vi "MainLUT.vi"(9 "Sample Number":u32, 10 "Run ID":string="run-1791786455269", 11 "LUT Selector":T3) -> (0 "error out":errorcluster, 3 "Sample":T1={"axis info"={"Horizontal"=0, "Vertical"=0, "Scrolling"=0}, "button info"={"button 1"=FALSE, "button 2"=FALSE, "button 3"=FALSE, "button 4"=FALSE}, "Relative Time (User Event)"=0.0, "Sample Number"=0, "Relative Time (Frame 0)"=0.0, "key mode"=enum."ABSOLUTE", "Frame Number"=0, "Keyboard KeysPressed"=[], "Keyboard No Op"=FALSE})   [LabVIEW 2026, in "dependencies.lvlib"]
uses:
  dependencies.lvlib
  KeyboardLUTSelector.ctl
  KeyboardAndMouseDataAcquisition.ctl
  KeyType.ctl
  ReplayMode.ctl
  RecordMode.ctl
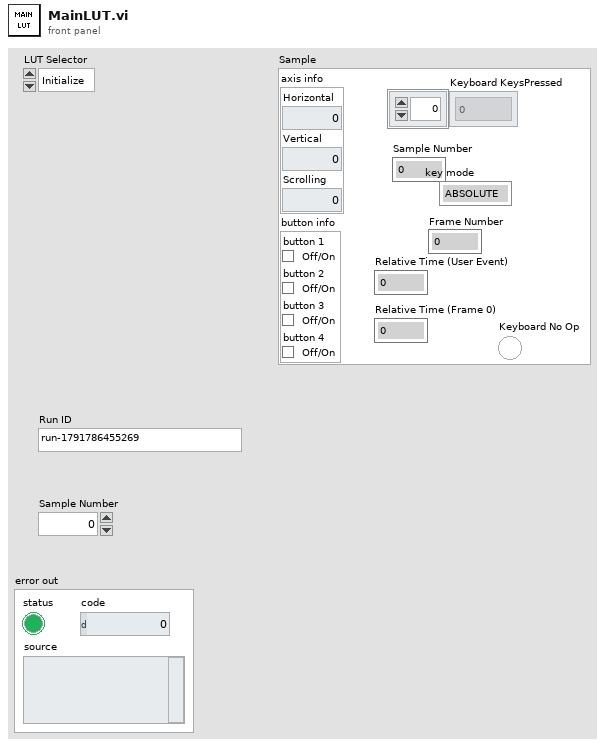
[diagram p1: front panel]
types:
  T1 = typedef "dependencies.lvlib/KeyboardAndMouseDataAcquisition.ctl" = cluster{"axis info":cluster{"Horizontal":i32, "Vertical":i32, "Scrolling":i32}, "button info":cluster{"button 1":bool, "button 2":bool, "button 3":bool, "button 4":bool}, "Relative Time (User Event)":dbl, "Sample Number":u32, "Relative Time (Frame 0)":dbl, "key mode":enum16{"RELATIVE", "ABSOLUTE"}, "Frame Number":u32, "Keyboard KeysPressed":T2[], "Keyboard No Op":bool}
  T2 = typedef "dependencies.lvlib/KeyType.ctl" = enum16{"0", "1", "2", "3", "4", "5", "6", "7", "8", "9", "A", "B", "C", "D", "E", "F", "G", "H", "I", "J", "K", "L", "M", "N", "O", "P", "Q", "R", "S", "T", "U", "V", "W", "X", "Y", "Z", "F1", "F2", "F3", "F4", "F5", "F6", "F7", "F8", "F9", "F10", "F11", "F12", "F13", "F14", "F15", "ADD", "BACK", "BACKSLASH", "CAPITAL", "COMMA", "DECIMAL", "DELETE", "DIVIDE", "DOWN", "END", "EQUALS", "ESCAPE", "GRAVE (`)", "HOME", "INSERT", "LBRACKET", "LCONTROL", "LEFT", "L ALT", "LSHIFT", "LWIN", "MINUS", "MULTIPLY", "NEXT", "NUMLOCK", "NUMPAD_0", "NUMPAD_1", "NUMPAD_2", "NUMPAD_3", "NUMPAD_4", "NUMPAD_5", "NUMPAD_6", "NUMPAD_7", "NUMPAD_8", "NUMPAD_9", "PAUSE", "PERIOD", "PRIOR (PG UP)", "RBRACKET", "RCONTROL", "RETURN", "RIGHT", "R ALT", "RSHIFT", "RWIN", "SCROLL", "SEMICOLON", "SLASH", "SPACE", "SUBTRACT", "TAB", "UP", "ENTER (num pad)", "' (quote)"}
  T3 = typedef "dependencies.lvlib/KeyboardLUTSelector.ctl" = enum16{"Initialize", "Get Keyboards Keys Pressed at Sample Number", "Assign Keyboard Key Press to Sample Number"}
  T4 = typedef "dependencies.lvlib/RecordMode.ctl" = enum16{"None", "User Events", "Benchmarks", "User Events and Benchmarks"}
  T5 = typedef "dependencies.lvlib/ReplayMode.ctl" = enum16{"None", "User Events"}
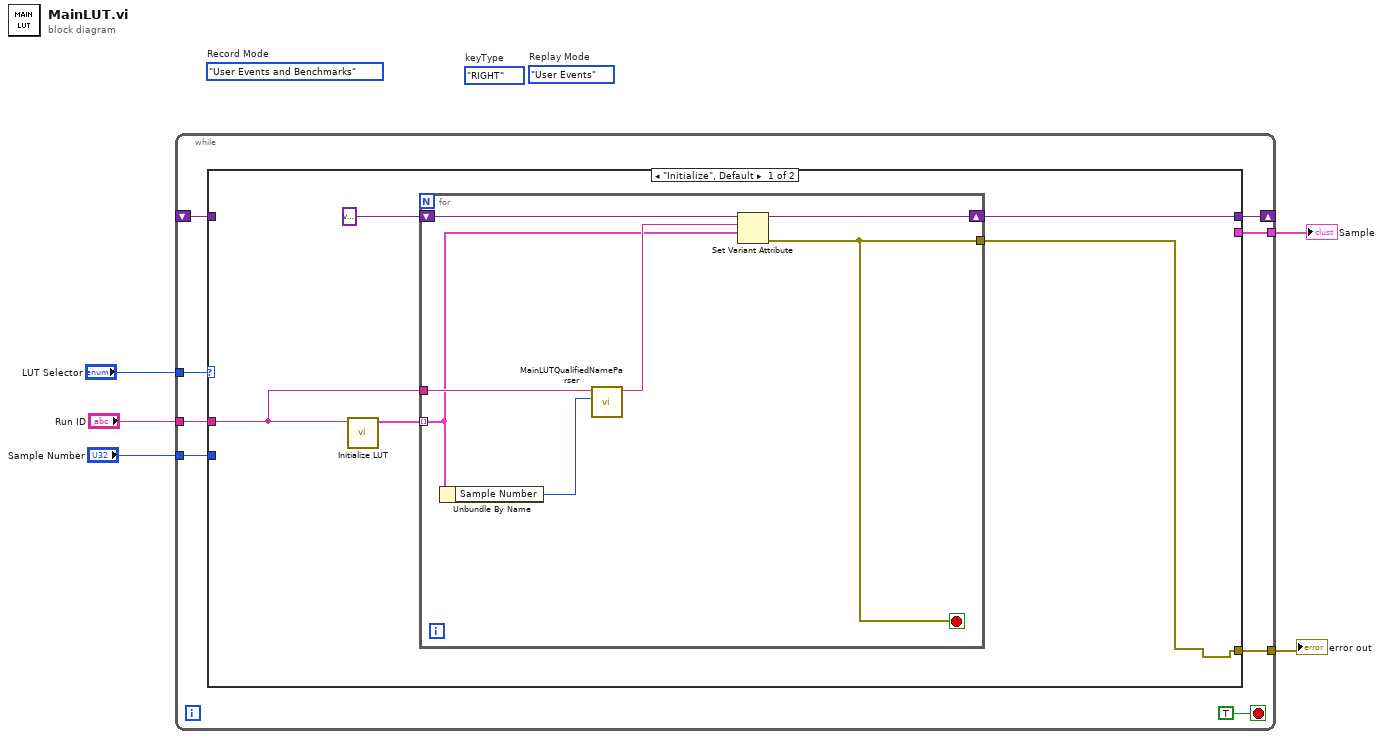
[diagram p0: block diagram]
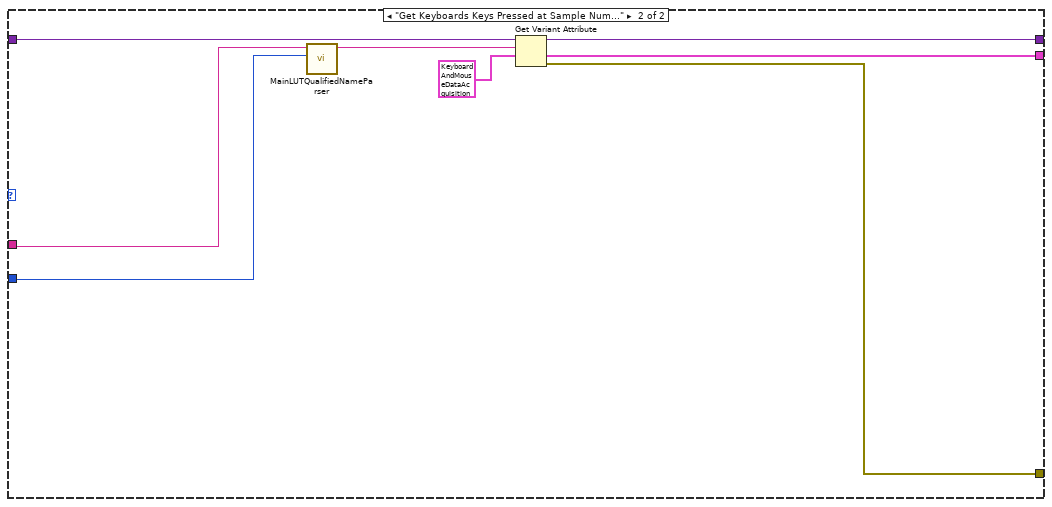
[diagram p2: hidden frame]
diagram:
  (unwired) RecordMode."User Events and Benchmarks"  # Record Mode
  (unwired) ReplayMode."User Events"  # Replay Mode
  (unwired) KeyType."RIGHT"  # keyType
  n1 = while {
    tunnel: "LUT Selector" -> [w12]
    shift-right: [w11] -> _
    shift-left: _ -> [w10]
    tunnel: "Run ID" -> [w9]
    tunnel: "Sample Number" -> [w8]
    tunnel: [w7] -> w1
    tunnel: [w6] -> w2
    stop <- TRUE stop-if-true
    n2 = case shown="\"Initialize\", Default" w12 {
      tunnel: [w15 w32] -> w11
      tunnel: w10 -> [_ w33]
      tunnel: w9 -> [w17 w31]
      tunnel: w8 -> [_ w30]
      tunnel: [_ w27] -> w7
      tunnel: [w14 w26] -> w6
      frame "Initialize", Default {
        n3 = call "Initialize LUT.vi"("Run ID"=w17) -> ("User Events Metadata"=w18:T1[])  [unwired: 10 in]
        n4 = for {
          tunnel: w18 -> [w20] mode=indexing
          tunnel: w17 -> [w25]
          shift-right: [w22] -> w15
          shift-left: variant -> [w23]
          tunnel: [w19] -> w14
          stop <- w19 stop-if-true
          n5 = Unbundle By Name(w20) -> ("Sample Number"=w24:u32)
          n6 = call "MainLUTQualifiedNameParser.vi"("Sample Number"=w24, "Run ID"=w25) -> ("QualifiedName"=w21:string)  [unwired: 9 in]
          n7 = Set Variant Attribute(Variant=w23, name=w21, value=w20) -> (Variant out=w22:variant, error out=w19:errorcluster)  [unwired: 1 in, 1 out]
        }
      }
      frame "Get Keyboards Keys Pressed at Sample Number" {
        n8 = call "MainLUTQualifiedNameParser.vi"("Sample Number"=w30, "Run ID"=w31) -> ("QualifiedName"=w29:string)  [unwired: 9 in]
        n9 = Get Variant Attribute(Variant=w33, name=w29, default value (empty Variant)=T1 {"axis info"={"Horizontal"=0, "Vertical"=0, "Scrolling"=0}, "button info"={"button 1"=FALSE, "button 2"=FALSE, "button 3"=FALSE, "button 4"=FALSE}, "Relative Time (User Event)"=0.0, "Sample Number"=0, "Relative Time (Frame 0)"=0.0, "key mode"=enum."ABSOLUTE", "Frame Number"=0, "Keyboard KeysPressed"=[], "Keyboard No Op"=FALSE} ("Data out")) -> (duplicate Variant=w32:variant, value=w27:T1, error out=w26:errorcluster)  [unwired: 1 in, 1 out]
      }
    }
  }
  "error out" <- w2
  "Sample" <- w1
